vi "Test Event Triggered.vi"(8 "error in":errorcluster, 10 "TestEvent":T1, 11 "Module ID":i32=-1) -> (0 "error out":errorcluster)   [LabVIEW 2026, in "UserEventRecorder.lvlib"]
doc: "_____\nCreated using DQMH Framework: Event Scripter 7.1.2.1547."
uses:
  UserEventRecorder.lvlib
  dependencies.lvlibp/dependencies/src/TestEvent.ctl
  Test Event Triggered Argument--cluster.ctl
  dependencies.lvlibp
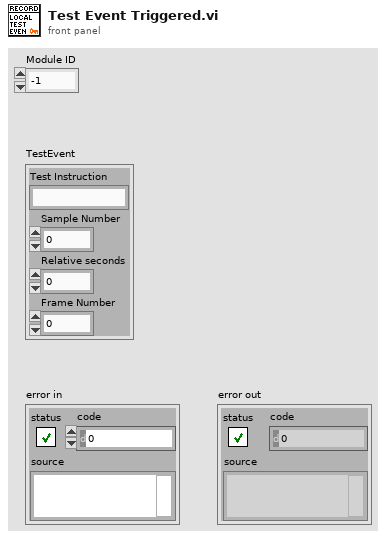
[diagram p1: front panel]
types:
  T1 = typedef "dependencies.lvlibp/TestEvent.ctl" = cluster{"Test Instruction":string, "Sample Number":u32, "Relative seconds":dbl, "Frame Number":u32}
  T2 = typedef "UserEventRecorder.lvlib/Test Event Triggered Argument--cluster.ctl" = cluster{"Module ID":i32, "TestEvent":T1}
  T3 = typedef "UserEventRecorder.lvlib/Request Events--cluster.ctl" = cluster{"Stop Module":refnum<user-event>, "Show Panel":refnum<user-event>, "Hide Panel":refnum<user-event>, "Show Diagram":refnum<user-event>, "Get Module Execution Status":refnum<user-event>, "Record Frame Mouse Metadata":refnum<user-event>, "Local Instance":T4}
  T4 = typedef "UserEventRecorder.lvlib/Local Instance Request Events--cluster.ctl" = cluster{"Test Event Triggered":refnum<user-event>}
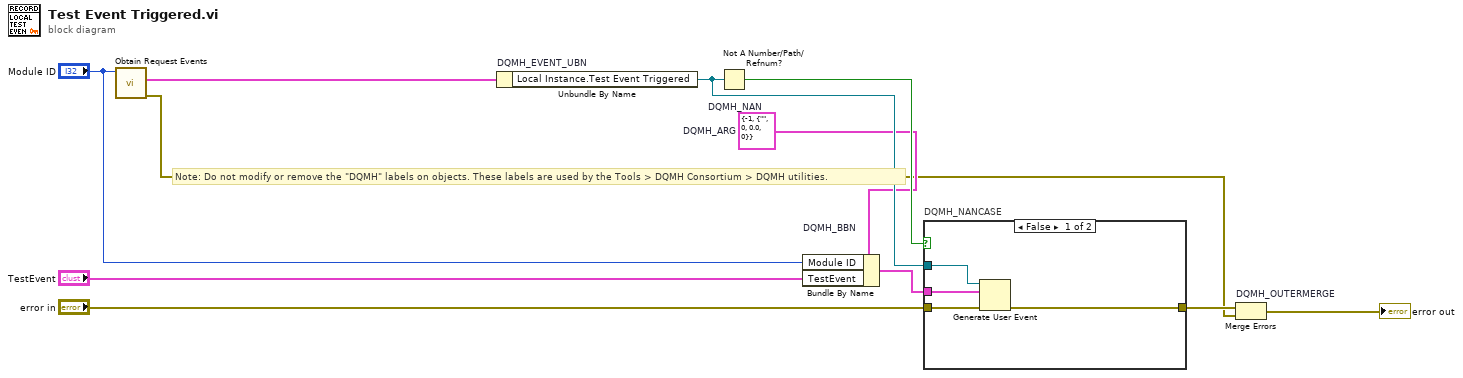
[diagram p0: block diagram]
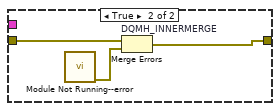
[diagram p2: hidden frame]
diagram:
  w5 = T2 {"Module ID"=-1, "TestEvent"={"Test Instruction"="", "Sample Number"=0, "Relative seconds"=0.0, "Frame Number"=0}}  # DQMH_ARG
  # "Note: Do not modify or remove the \"DQMH\" labels on objects. These labels are used by the Tools > DQMH Consortium > DQMH utilities."
  n1 = call "Obtain Request Events.vi"("Module ID"="Module ID") -> ("error out"=w2:errorcluster, "UserEventRecorder Request Events"=w1:T3)  [unwired: 9 in]
  n2 = Unbundle By Name "DQMH_EVENT_UBN"(w1) -> ("Local Instance.Test Event Triggered"=w7:refnum<user-event>)
  n3 = Not A Number/Path/Refnum? "DQMH_NAN"(number/path/refnum=w7) -> (NaN/Path/Refnum?=w8:bool)
  n4 = Bundle By Name "DQMH_BBN"(cluster=w5, "Module ID"="Module ID", "TestEvent"="TestEvent") -> (w9:T2)
  n5 = case "DQMH_NANCASE" shown="False" w8 {
    tunnel: "error in" -> [w15 w18]
    tunnel: [w14 w17] -> w6
    tunnel: w7 -> [w13 _]
    tunnel: w9 -> [w12 _]
    frame False {
      n6 = Generate User Event(user event=w13, event data cluster=w12, error in=w15) -> (error out=w14:errorcluster)  [unwired: 1 in, 1 out]
    }
    frame True {
      n7 = call "Module Not Running--error.vi"() -> ("error out"=w16:errorcluster)  [unwired: 11 in]
      n8 = Merge Errors "DQMH_INNERMERGE"(w18, w16) -> (w17:errorcluster)
    }
  }
  n9 = Merge Errors "DQMH_OUTERMERGE"(w6, w2) -> (→"error out":errorcluster)
